vi "Test BB write read.vi"() -> ()   [LabVIEW 2021]
uses:
  typedef/Topic Full Names.ctl
  fc94ccf3-c4f9-4681-abcb-997b10467b18.vi
  1ecc9c55-0292-4034-a41c-db8078422293.vi
  9e8af28e-348a-4d52-b3a6-176f81345950.vi
  ff93d857-b347-4659-b587-d301aa5bbc46.vi
  d7d53fbf-e9ea-4da0-a5dc-3f6decd5c89f.vi
  386e704e-7c72-4735-ad53-a1b4597bfffc.vi
  aea694b6-2c48-4883-b1e6-448c91e8bea0.vi
  af7b2d98-0160-47b9-b2c8-6d5a41cd72f1.vi
  04c724ed-f4c4-49d6-b90b-59eac79b411c.vi
  10f2c807-d207-4ff9-b65f-d1b3e01e3914.vi
  96694315-c729-49e0-ae38-07976d2b01df.vi
  07ed32da-fde3-4ecc-a422-c66c6e158a99.vi
  5cbece44-eccb-42af-b590-0ccb7b3e0a3a.vi
  26da49ab-0f24-4915-9e5c-fae2186c0621.vi
  82d32cb3-3716-468c-9992-8dfaf92fc29f.vi
  0ce00b95-44ee-463c-baca-590a8846c1eb.vi
  5a159916-ffba-4323-afb6-8e2cf34b4672.vi
  0118180c-ae51-4c1e-a806-e67c93401480.vi
  9acccfa8-9bb2-4941-a38e-bb205dd59574.vi
  ab6a61a5-9c5f-449d-8423-f873c584b1ba.vi
  540d5d61-12e3-498b-9d40-879b6436794c.vi
  17e3f022-6cbe-4307-a055-1088f1a08aa5.vi
  b63f9921-ff80-4853-b2dc-f0cfe3ce2752.vi
  df38f484-dfd4-40f9-b9a1-491e45d6069d.vi
  dabef161-ca45-40be-b185-d2158fafdac9.vi
  599458bd-4083-4966-a6e9-0ee856bb8018.vi
  f13160dd-4d28-4d65-9fc8-a661e616088f.vi
  2429a5ee-c682-4303-b56b-a50622380fa0.vi
  c451a5a5-bbd7-4334-95d0-190131a98318.vi
  4afb852e-2286-42e1-bd7d-983000913123.vi
  c331ddf7-6c60-4b7b-82e2-165266058c85.vi
  989f7903-0cec-405a-8fc5-4e05a1e3b823.vi
  3f8d1f86-cf74-40ec-b4a0-b5d2f462e92c.vi
  c2603ed1-ff0f-47d7-9edf-26bf5f6ef7d4.vi
  9dc61f32-c8b2-401f-b4c2-5e38d3c4ff08.vi
  f2a7571f-032b-4f55-a724-f4471c08458c.vi
  dc893c51-4d2e-4bb4-b285-f4d4203b9537.vi
  91a0fbaa-2358-4159-8e72-b3850ae0b459.vi
  54bee8c1-0067-4be9-af3e-190d85fa807a.vi
  b4ab5d2e-a320-4709-8a65-b849ff6d5eac.vi
  c90ed56e-a4fb-44b1-b21c-7cee833b7fc2.vi
  8dfab18a-ac58-41df-a961-e3b183f267b1.vi
  6d6d06d4-fd38-4af0-8f86-16f866c4358f.vi
  70f752b6-94b3-46bc-87c5-c5551f755e49.vi
  87693e93-dc1b-4689-9420-073608a864a2.vi
  d23bcab6-9216-4072-ab24-334b80493afe.vi
  13594309-f9d5-44d8-84db-906724c8aeb8.vi
  5b121a18-a7f8-444b-bf3c-19de00dea731.vi
  b678fec2-0823-4dac-b98e-1ea96459124d.vi
  421e2864-b975-4d6e-8dba-970c1d659c6b.vi
  83d6945f-6206-48db-ba34-1315ddcf8622.vi
  334fafdd-3c45-415d-86a5-5c46786f1213.vi
  bdeeffe2-7481-4f0c-a63b-1c279b4d539b.vi
  daf0490c-48a1-49ff-a818-56076b47f53a.vi
  6d140309-082e-4568-9266-a5523fd3356c.vi
  cd00a663-0ed0-4c1c-bf6f-1e92360d99b7.vi
  0e6f1a11-abca-4238-a699-ce8b92277205.vi
  08820cd5-e149-4070-b260-5d58bdcecb90.vi
  8688fec4-49dd-4baa-ba4f-355704276364.vi
  62f858e5-9e8a-46a7-a3e9-f0995d3fb264.vi
  08794ecb-60ec-43ee-b589-61fe16b07a23.vi
  29a63749-4c43-41a6-a3ab-cfd97f2cae72.vi
  19342fc4-a6b3-4ce5-a15c-c0c74d8c0e55.vi
  0190af3f-4f2e-4064-95c6-6e90d87b853f.vi
  c9e0bfd6-1a21-40a0-b211-991072438108.vi
  849b2bb5-713d-46b1-af3e-8376bcd0ab32.vi
  SubVIs/Get Path.vi
  SubVIs/Convert Error.vi
  fc94ccf3-c4f9-4681-abcb-997b10467b18.vi/f164bb55-fadc-406a-97d8-e3295a396b46.vi
  SubVIs/Add Error.vi
  Refnum/BB from Refnum.vi
  Refnum/BB Writer to Refnum.vi
  <vilib>/CIF Foundation/CIF Utilities/File/File/File Not Found Error Update.vi
  1ecc9c55-0292-4034-a41c-db8078422293.vi/15451e88-64ef-462d-9cc0-58968935b893.vi
  Refnum/BB Reader to Refnum.vi
  Refnum/BB Writer from Refnum.vi
  Refnum/BB Reader from Refnum.vi
  386e704e-7c72-4735-ad53-a1b4597bfffc.vi/f164bb55-fadc-406a-97d8-e3295a396b46.vi
  aea694b6-2c48-4883-b1e6-448c91e8bea0.vi/15451e88-64ef-462d-9cc0-58968935b893.vi
  96694315-c729-49e0-ae38-07976d2b01df.vi/3bd89bd1-b605-4b55-aa60-227046f12b11.vi
  07ed32da-fde3-4ecc-a422-c66c6e158a99.vi/bd005753-9160-49ee-ba23-7aa8055d86ff.vi
  0ce00b95-44ee-463c-baca-590a8846c1eb.vi/3bd89bd1-b605-4b55-aa60-227046f12b11.vi
  5a159916-ffba-4323-afb6-8e2cf34b4672.vi/bd005753-9160-49ee-ba23-7aa8055d86ff.vi
  540d5d61-12e3-498b-9d40-879b6436794c.vi/f164bb55-fadc-406a-97d8-e3295a396b46.vi
  17e3f022-6cbe-4307-a055-1088f1a08aa5.vi/15451e88-64ef-462d-9cc0-58968935b893.vi
  f13160dd-4d28-4d65-9fc8-a661e616088f.vi/f164bb55-fadc-406a-97d8-e3295a396b46.vi
  2429a5ee-c682-4303-b56b-a50622380fa0.vi/15451e88-64ef-462d-9cc0-58968935b893.vi
  3f8d1f86-cf74-40ec-b4a0-b5d2f462e92c.vi/f164bb55-fadc-406a-97d8-e3295a396b46.vi
  c2603ed1-ff0f-47d7-9edf-26bf5f6ef7d4.vi/15451e88-64ef-462d-9cc0-58968935b893.vi
  dc893c51-4d2e-4bb4-b285-f4d4203b9537.vi/f164bb55-fadc-406a-97d8-e3295a396b46.vi
  91a0fbaa-2358-4159-8e72-b3850ae0b459.vi/15451e88-64ef-462d-9cc0-58968935b893.vi
  c90ed56e-a4fb-44b1-b21c-7cee833b7fc2.vi/f164bb55-fadc-406a-97d8-e3295a396b46.vi
  8dfab18a-ac58-41df-a961-e3b183f267b1.vi/15451e88-64ef-462d-9cc0-58968935b893.vi
  87693e93-dc1b-4689-9420-073608a864a2.vi/3bd89bd1-b605-4b55-aa60-227046f12b11.vi
  Refnum/BB Raw Reader to Refnum.vi
  Refnum/BB Raw Reader from Refnum.vi
  13594309-f9d5-44d8-84db-906724c8aeb8.vi/c28b0ead-42ad-4072-80a2-aca7f2bd7ce3.vi
  13594309-f9d5-44d8-84db-906724c8aeb8.vi/48104490-ec73-4168-8754-ff252ec03617.vi
  <vilib>/CIF Foundation/CIF Utilities/DataTypes/SubVIs/DataTypes Error.vi
  13594309-f9d5-44d8-84db-906724c8aeb8.vi/543c0f61-77eb-4f29-b175-1688c1700ba4.vi
  b678fec2-0823-4dac-b98e-1ea96459124d.vi/f164bb55-fadc-406a-97d8-e3295a396b46.vi
  421e2864-b975-4d6e-8dba-970c1d659c6b.vi/15451e88-64ef-462d-9cc0-58968935b893.vi
  daf0490c-48a1-49ff-a818-56076b47f53a.vi/f164bb55-fadc-406a-97d8-e3295a396b46.vi
  6d140309-082e-4568-9266-a5523fd3356c.vi/15451e88-64ef-462d-9cc0-58968935b893.vi
  8688fec4-49dd-4baa-ba4f-355704276364.vi/f164bb55-fadc-406a-97d8-e3295a396b46.vi
  62f858e5-9e8a-46a7-a3e9-f0995d3fb264.vi/3bd89bd1-b605-4b55-aa60-227046f12b11.vi
  08794ecb-60ec-43ee-b589-61fe16b07a23.vi/bd005753-9160-49ee-ba23-7aa8055d86ff.vi
  Refnum/BB Raw Writer to Refnum.vi
  Refnum/BB Raw Writer from Refnum.vi
  <vilib>/Utility/error.llb/Trim Whitespace.vi
  SubVIs/Add Error Core.vi
  <vilib>/CIF Foundation/CIF Utilities/DataTypes/Utilities/Get Element Info of Variant.vi
  SubVIs/Get Type String.vi
  <vilib>/CIF Foundation/CIF Utilities/DataTypes/Utilities/Get JSON Descriptor of Variant.vi
  SubVIs/Convert Error Core.vi
  <vilib>/CIF Foundation/CIF Utilities/File/SubVIs/File Not Found Error Core.vi
  <vilib>/CIF Foundation/CIF Utilities/DataTypes/SubVIs/DataTypes Error Core.vi
  Iceoryx.lvlib
panel:
  out "status":string
  out "pass":bool
  out "error out":errorcluster
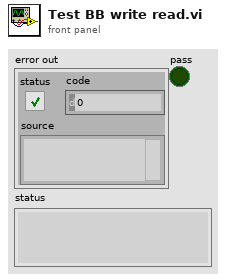
[diagram p1: front panel]
types:
  T1 = typedef "Iceoryx.lvlib/Topic Full Names.ctl" = cluster{"BlackBoard":string, "Topic":string, "Type Override":string}
  T2 = cluster{"U16":u16, "test_I32":i32, bool, "embedded":cluster{dbl, "bool":bool}}
  T3 = typedef "Iceoryx.lvlib/BB Refnum.ctl" = cluster{"refnum":u64, "BB":enum8{"bb"}}
  T4 = typedef "Iceoryx.lvlib/BB Writer Refnum.ctl" = cluster{"refnum":u64, "BB Writer":enum8{"bb_writer"}}
  T5 = typedef "Iceoryx.lvlib/BB Reader Refnum.ctl" = cluster{"refnum":u64, "BB Reader":enum8{"bb_reader"}}
  T6 = cluster{"U16":u16, "I32":i32, bool, "embedded":cluster{dbl, "bool":bool}}
  T7 = typedef "Iceoryx.lvlib/BB Raw Reader Refnum.ctl" = cluster{"refnum":u64, "BB Raw Reader":enum8{"bb_raw_reader"}}
  T8 = typedef "Iceoryx.lvlib/BB Raw Writer Refnum.ctl" = cluster{"refnum":u64, "BB Raw Writer":enum8{"bb_raw_writer"}}
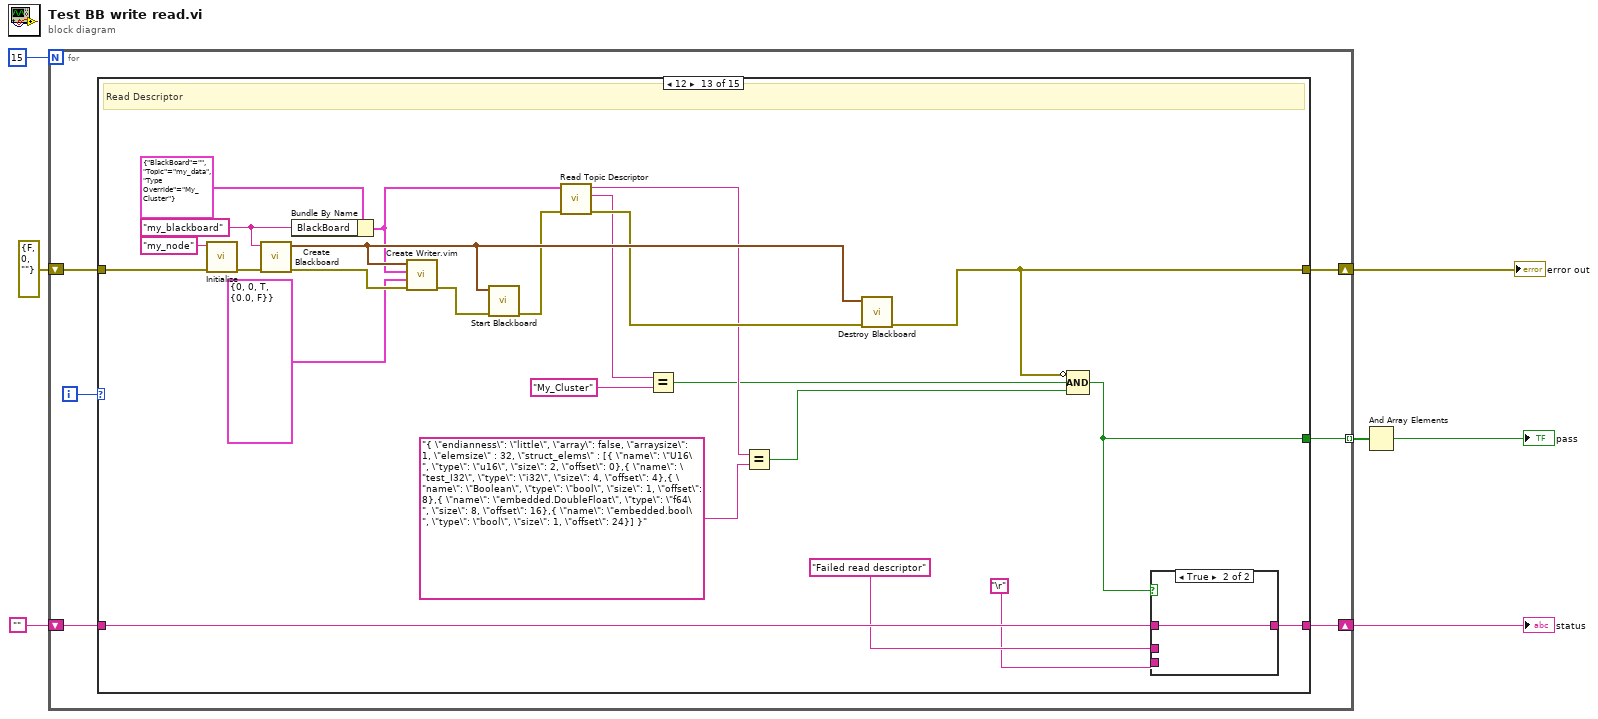
[diagram p0: block diagram]
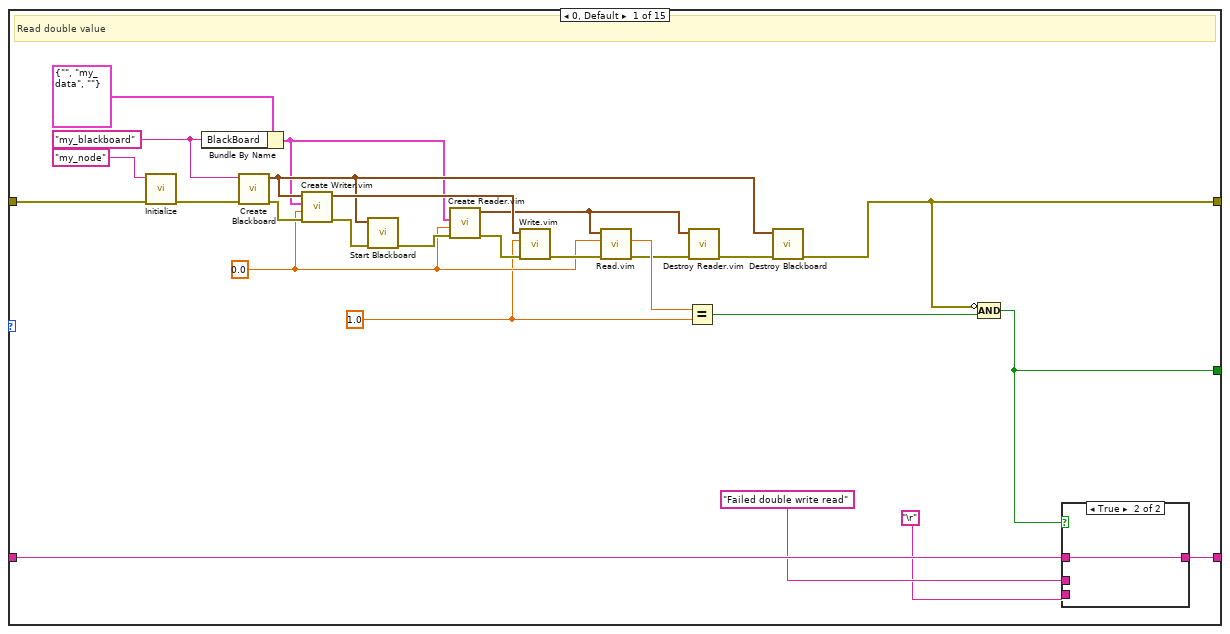
[diagram p2: hidden frame]
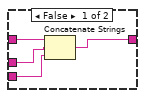
[diagram p3: hidden frame]
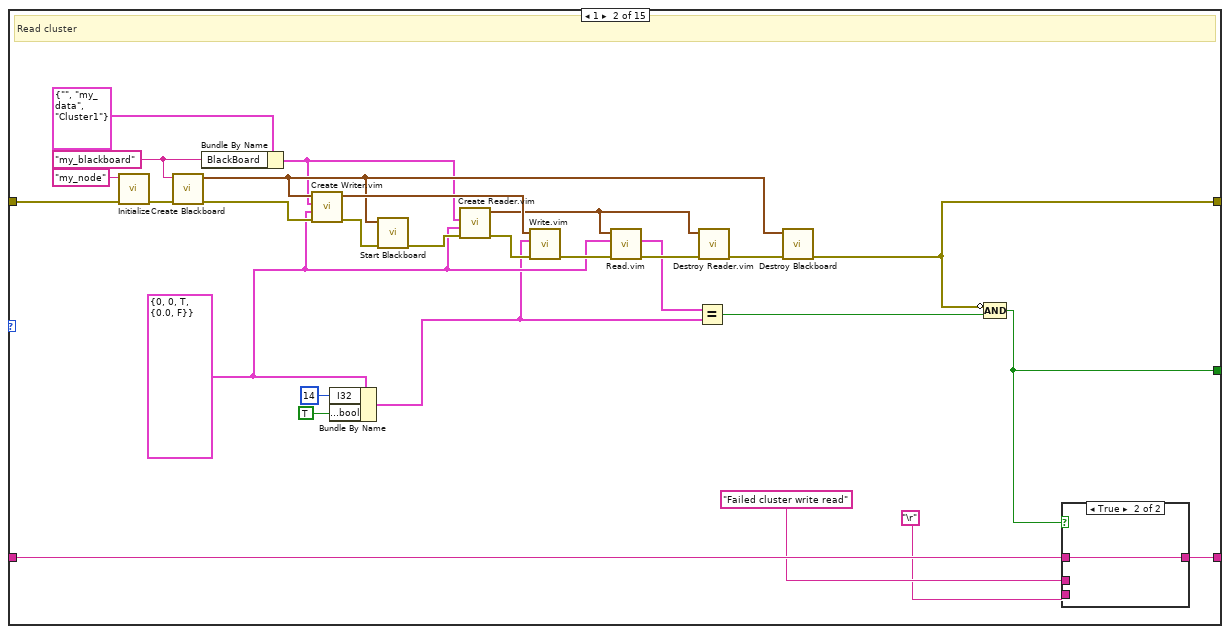
[diagram p4: hidden frame]
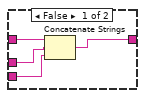
[diagram p5: hidden frame]
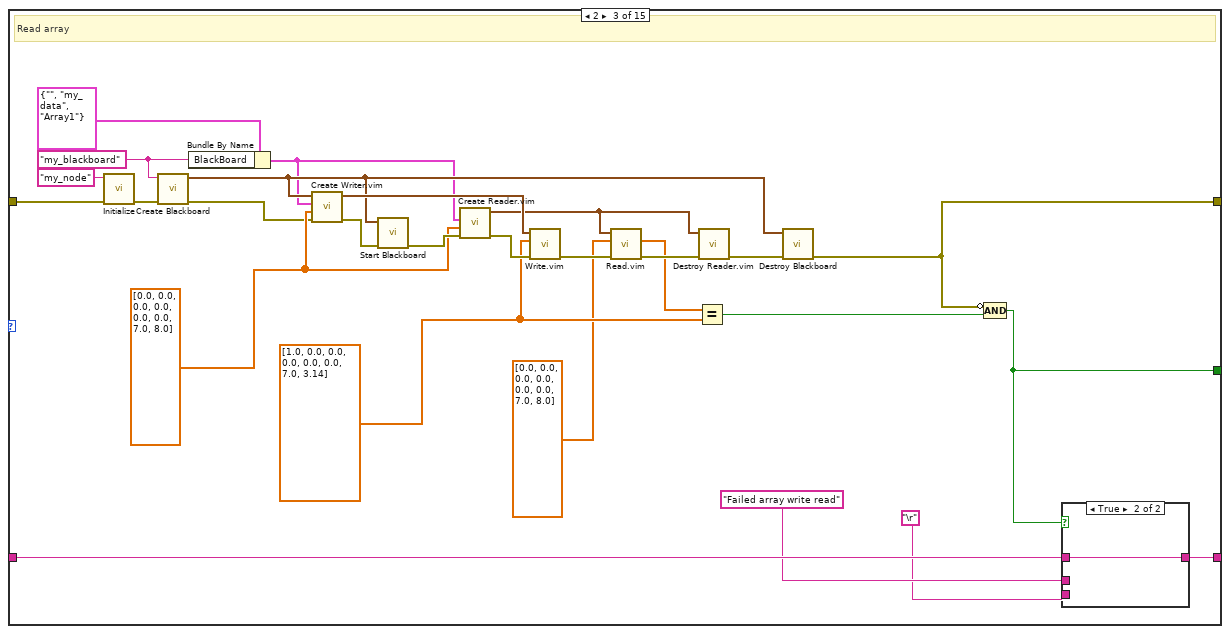
[diagram p6: hidden frame]
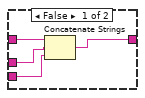
[diagram p7: hidden frame]
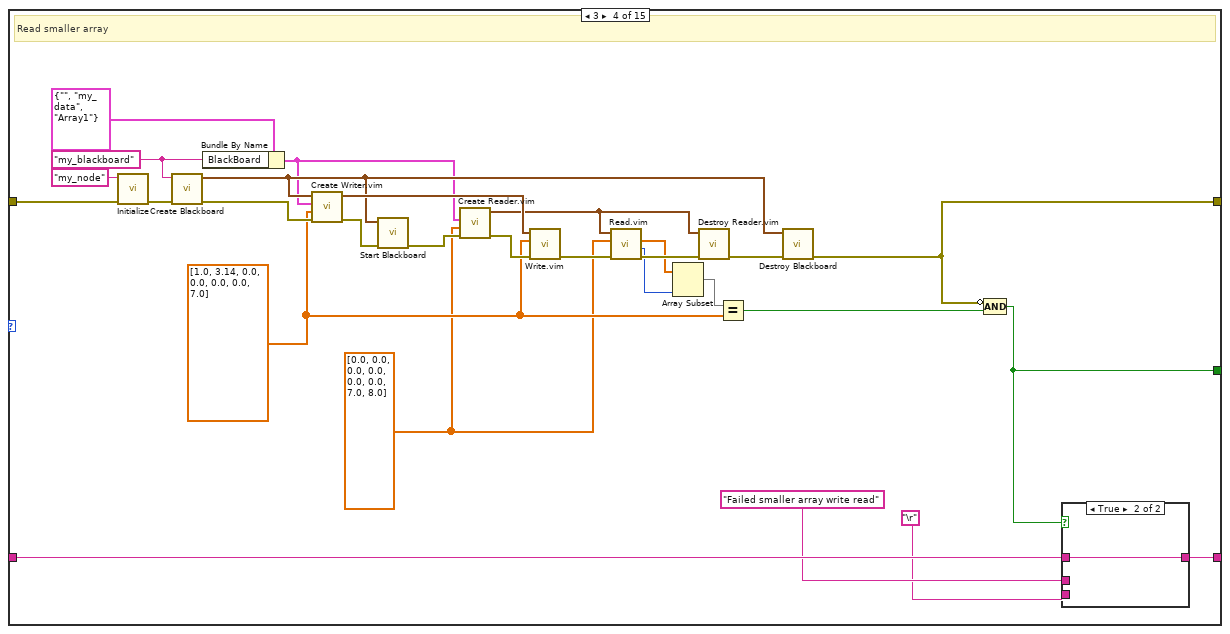
[diagram p8: hidden frame]
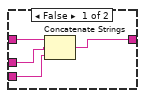
[diagram p9: hidden frame]
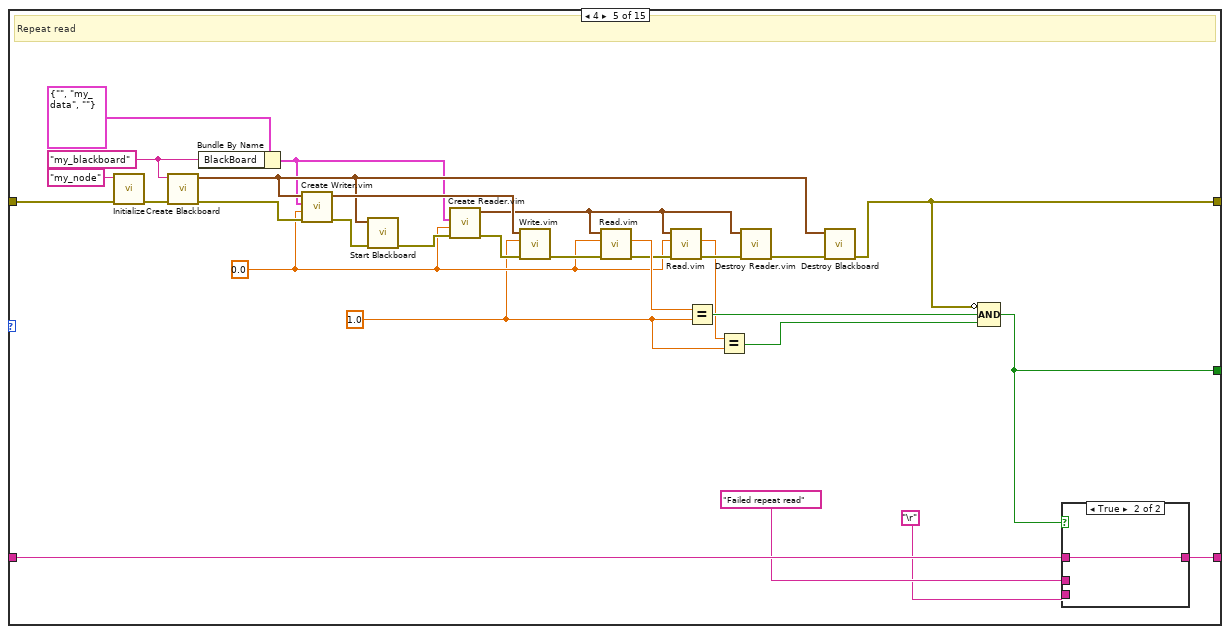
[diagram p10: hidden frame]
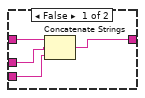
[diagram p11: hidden frame]
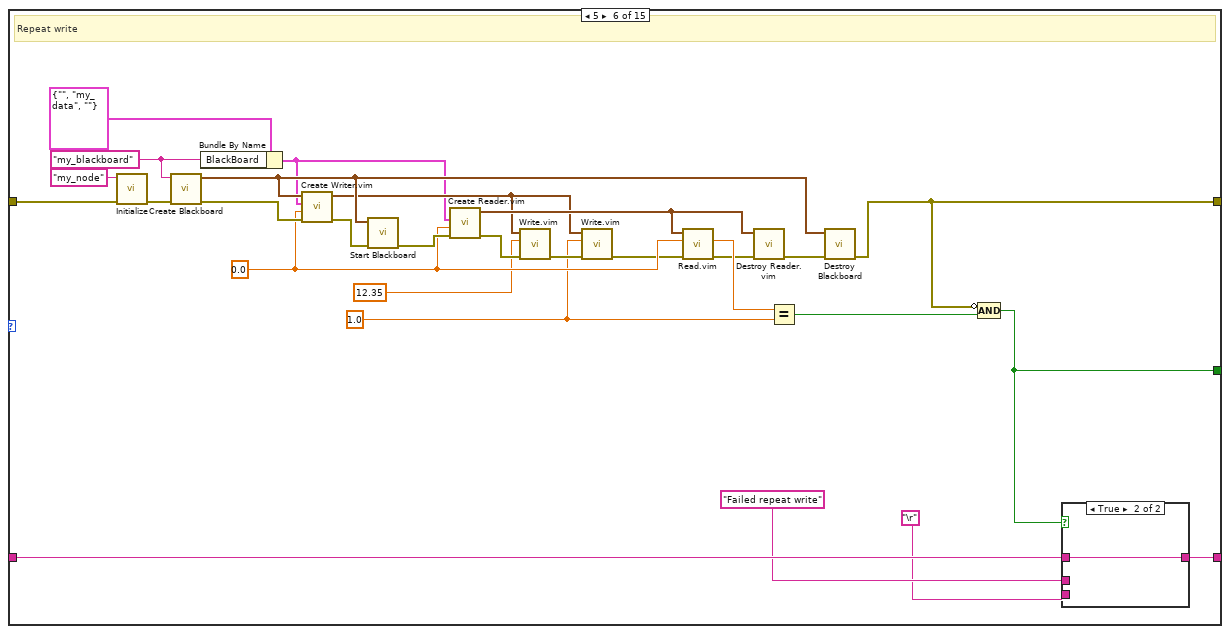
[diagram p12: hidden frame]
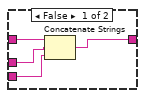
[diagram p13: hidden frame]
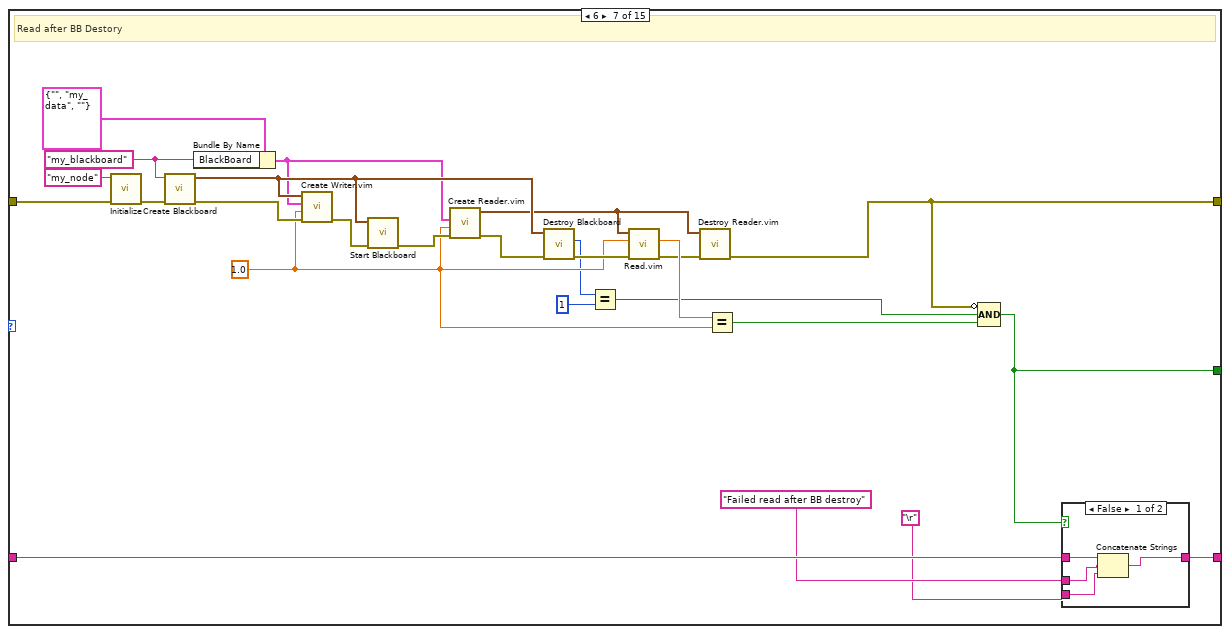
[diagram p14: hidden frame]
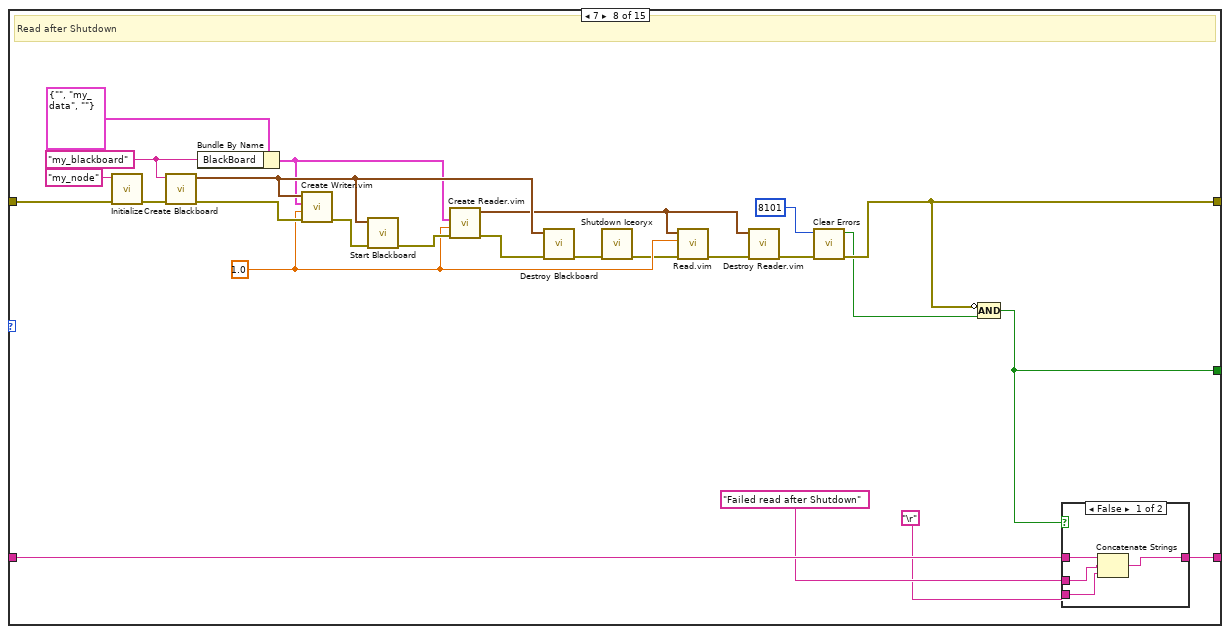
[diagram p16: hidden frame]
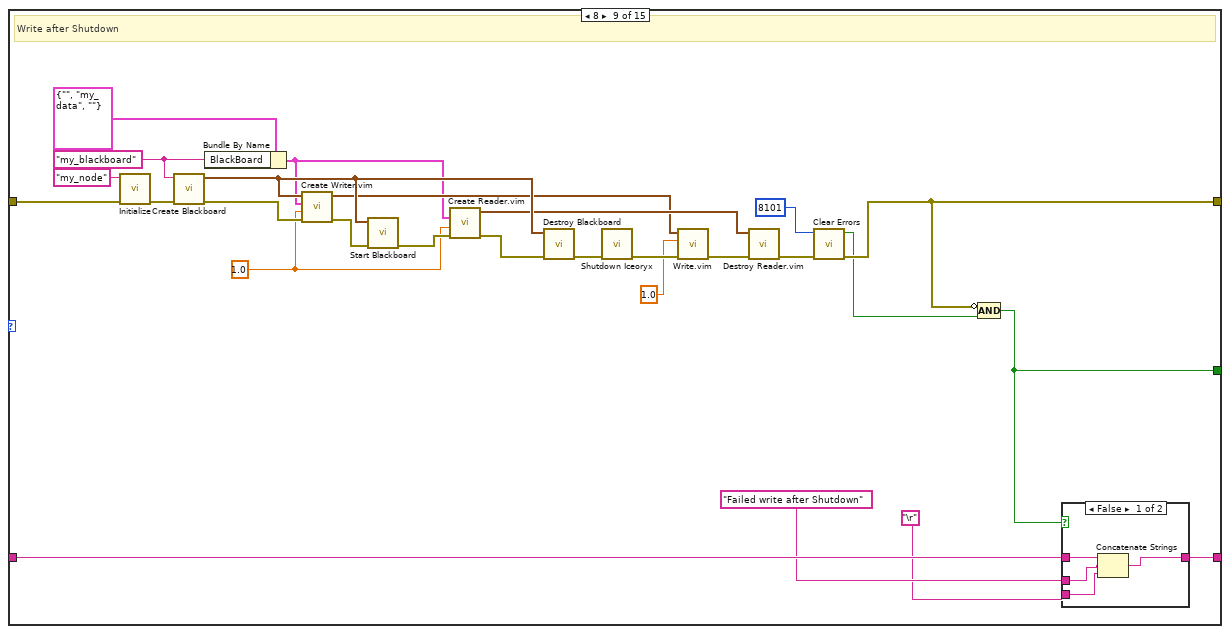
[diagram p18: hidden frame]
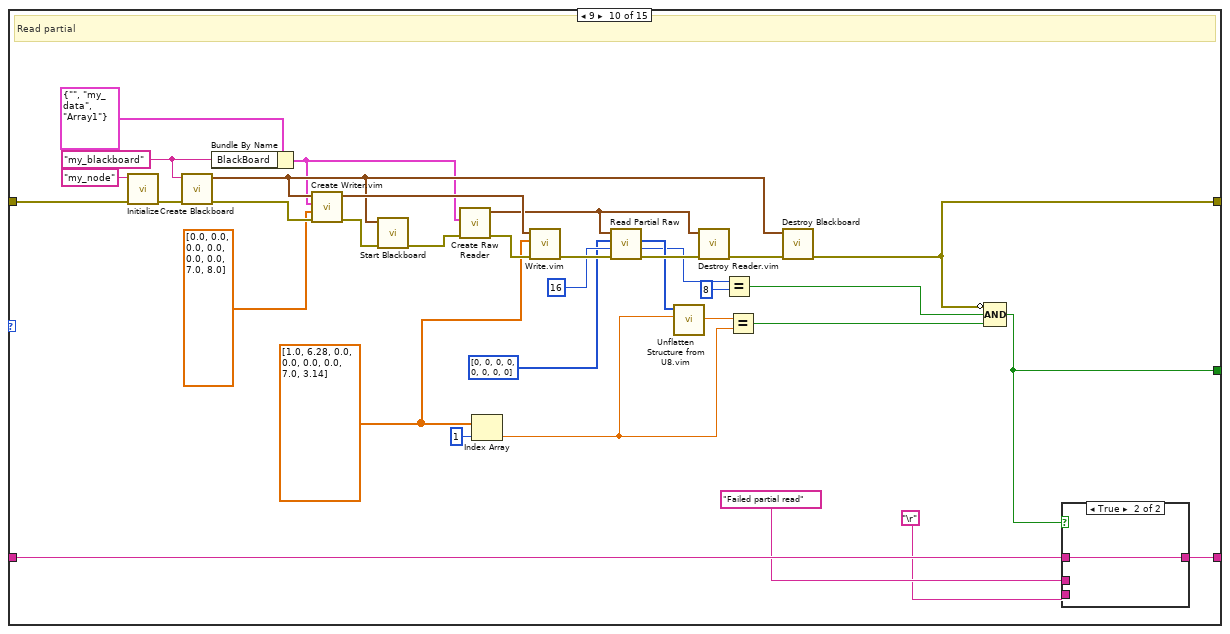
[diagram p20: hidden frame]
diagram:
  n1 = for {
    N: 15 -> [_]
    tunnel: [w13] -> w7 mode=indexing
    shift-right: [w11] -> w3
    shift-left: "" -> [w12]
    shift-right: [w10] -> w1
    shift-left: errorcluster {"status"=FALSE, "code"=0, "source"=""} ("error out") -> [w9]
    i -> [w8]
    n2 = case shown="12" w8 {
      tunnel: [w35 w48 w86 w118 w167 w200 w231 w261 w293 w318 w366 w403 w432 w458 w485] -> w13
      tunnel: w12 -> [w39 w72 w104 w137 w171 w204 w235 w265 w297 w336 w370 w407 w436 w471 w503]
      tunnel: [w38 w71 w103 w136 w170 w203 w234 w264 w296 w335 w369 w406 w435 w470 w502] -> w11
      tunnel: [w19 w53 w87 w119 w153 w188 w219 w246 w278 w319 w350 w389 w425 w459 w486] -> w10
      tunnel: w9 -> [w32 w54 w88 w120 w164 w197 w229 w259 w291 w320 w363 w400 w430 w460 w487]
      frame 0, Default {
        w21 = 0.0
        w14 = 1.0
        w16 = "my_blackboard" ("Blackboard name")
        # "Read double value"
        n3 = call "Initialize.vi"("error in (no error)"=w32, "Node name"="my_node") -> ("error out"=w33:errorcluster)  [unwired: 9 in]
        n4 = Bundle By Name(cluster=T1 {"BlackBoard"="", "Topic"="my_data", "Type Override"=""} ("Topic Full Names"), "BlackBoard"=w16) -> (w15:T1)
        n5 = call "Create Blackboard.vi"("error in (no error)"=w33, "Blackboard name"=w16) -> ("error out"=w30:errorcluster, "Blackboard Reference"=w22:T3)  [unwired: 8 in]
        n6 = call "Create Writer.vim"("error in (no error)"=w30, "Data"=w21, "Topic Name"=w15, "BlackBoard Reference"=w22) -> ("error out"=w31:errorcluster, "Writer Reference"=w24:T4)  [unwired: 5 in, 1 out]
        n7 = call "Start Blackboard.vi"("error in (no error)"=w31, "Blackboard Reference"=w22) -> ("error out"=w29:errorcluster)  [unwired: 9 in]
        n8 = call "Create Reader.vim"("error in (no error)"=w29, "Data Type"=w21, "Topic Name"=w15) -> ("error out"=w28:errorcluster, "Reader Reference"=w23:T5)  [unwired: 6 in, 1 out]
        n9 = call "Write.vim"("error in (no error)"=w28, "Data In"=w14, "Writer Reference"=w24) -> ("error out"=w27:errorcluster)  [unwired: 7 in, 1 out]
        n10 = call "Read.vim"("error in (no error)"=w27, "Data In"=w21, "Reader Reference"=w23) -> ("error out"=w17:errorcluster, "Data Out"=w20:dbl)  [unwired: 6 in, 1 out]
        n11 = Equal?(x=w20, y=w14) -> (x = y?=w34:bool)
        n12 = call "Destroy Reader.vim"("error in (no error)"=w17, "Reader Reference"=w23) -> ("error out"=w26:errorcluster)  [unwired: 9 in]
        n13 = call "Destroy Blackboard.vi"("error in (no error)"=w26, "Blackboard Reference"=w22) -> ("error out"=w19:errorcluster)  [unwired: 8 in, 1 out]
        n14 = Compound Arithmetic op=AND(invert w19, w34) -> (w35:bool)
        n15 = case shown="True" w35 {
          tunnel: w39 -> [w43 w44]
          tunnel: [w40 w44] -> w38
          tunnel: "Failed double write read" -> [w42 _]
          tunnel: "\r" -> [w41 _]
          frame False {
            n16 = Concatenate Strings(w43, w42, w41) -> (w40:string)
          }
          frame True {
          }
        }
      }
      frame 1 {
        w50 = T6 {"U16"=0, "I32"=0, TRUE, "embedded"={0.0, "bool"=FALSE}}
        w47 = "my_blackboard" ("Blackboard name")
        # "Read cluster"
        n17 = call "Initialize.vi"("error in (no error)"=w54, "Node name"="my_node") -> ("error out"=w67:errorcluster)  [unwired: 9 in]
        n18 = call "Create Blackboard.vi"("error in (no error)"=w67, "Blackboard name"=w47) -> ("error out"=w65:errorcluster, "Blackboard Reference"=w56:T3)  [unwired: 8 in]
        n19 = Bundle By Name(cluster=T1 {"BlackBoard"="", "Topic"="my_data", "Type Override"="Cluster1"} ("Topic Full Names"), "BlackBoard"=w47) -> (w45:T1)
        n20 = call "Create Writer.vim"("error in (no error)"=w65, "Data"=w50, "Topic Name"=w45, "BlackBoard Reference"=w56) -> ("error out"=w66:errorcluster, "Writer Reference"=w58:T4)  [unwired: 5 in, 1 out]
        n21 = Bundle By Name(cluster=w50, "I32"=14, "embedded.bool"=TRUE) -> (w49:T6)
        n22 = call "Start Blackboard.vi"("error in (no error)"=w66, "Blackboard Reference"=w56) -> ("error out"=w64:errorcluster)  [unwired: 9 in]
        n23 = call "Create Reader.vim"("error in (no error)"=w64, "Data Type"=w50, "Topic Name"=w45) -> ("error out"=w63:errorcluster, "Reader Reference"=w57:T5)  [unwired: 6 in, 1 out]
        n24 = call "Write.vim"("error in (no error)"=w63, "Data In"=w49, "Writer Reference"=w58) -> ("error out"=w62:errorcluster)  [unwired: 7 in, 1 out]
        n25 = call "Read.vim"("error in (no error)"=w62, "Data In"=w50, "Reader Reference"=w57) -> ("error out"=w61:errorcluster, "Data Out"=w55:T6)  [unwired: 6 in, 1 out]
        n26 = Equal?(x=w55, y=w49) -> (x = y?=w68:bool)
        n27 = call "Destroy Reader.vim"("error in (no error)"=w61, "Reader Reference"=w57) -> ("error out"=w60:errorcluster)  [unwired: 9 in]
        n28 = call "Destroy Blackboard.vi"("error in (no error)"=w60, "Blackboard Reference"=w56) -> ("error out"=w53:errorcluster)  [unwired: 8 in, 1 out]
        n29 = Compound Arithmetic op=AND(invert w53, w68) -> (w48:bool)
        n30 = case shown="True" w48 {
          tunnel: w72 -> [w76 w77]
          tunnel: [w73 w77] -> w71
          tunnel: "Failed cluster write read" -> [w75 _]
          tunnel: "\r" -> [w74 _]
          frame False {
            n31 = Concatenate Strings(w76, w75, w74) -> (w73:string)
          }
          frame True {
          }
        }
      }
      frame 2 {
        w84 = dbl[] [1.0, 0.0, 0.0, 0.0, 0.0, 0.0, 7.0, 3.14]
        w85 = dbl[] [0.0, 0.0, 0.0, 0.0, 0.0, 0.0, 7.0, 8.0]
        w80 = "my_blackboard" ("Blackboard name")
        # "Read array"
        n32 = call "Initialize.vi"("error in (no error)"=w88, "Node name"="my_node") -> ("error out"=w99:errorcluster)  [unwired: 9 in]
        n33 = call "Create Blackboard.vi"("error in (no error)"=w99, "Blackboard name"=w80) -> ("error out"=w79:errorcluster, "Blackboard Reference"=w89:T3)  [unwired: 8 in]
        n34 = Bundle By Name(cluster=T1 {"BlackBoard"="", "Topic"="my_data", "Type Override"="Array1"} ("Topic Full Names"), "BlackBoard"=w80) -> (w78:T1)
        n35 = call "Create Writer.vim"("error in (no error)"=w79, "Data"=w85, "Topic Name"=w78, "BlackBoard Reference"=w89) -> ("error out"=w98:errorcluster, "Writer Reference"=w91:T4)  [unwired: 5 in, 1 out]
        n36 = call "Start Blackboard.vi"("error in (no error)"=w98, "Blackboard Reference"=w89) -> ("error out"=w97:errorcluster)  [unwired: 9 in]
        n37 = call "Create Reader.vim"("error in (no error)"=w97, "Data Type"=w85, "Topic Name"=w78) -> ("error out"=w96:errorcluster, "Reader Reference"=w90:T5)  [unwired: 6 in, 1 out]
        n38 = call "Write.vim"("error in (no error)"=w96, "Data In"=w84, "Writer Reference"=w91) -> ("error out"=w95:errorcluster)  [unwired: 7 in, 1 out]
        n39 = call "Read.vim"("error in (no error)"=w95, "Data In"=dbl[] [0.0, 0.0, 0.0, 0.0, 0.0, 0.0, 7.0, 8.0], "Reader Reference"=w90) -> ("error out"=w94:errorcluster, "Data Out"=w83:dbl[])  [unwired: 6 in, 1 out]
        n40 = Equal?(x=w83, y=w84) -> (x = y?=w100:bool)
        n41 = call "Destroy Reader.vim"("error in (no error)"=w94, "Reader Reference"=w90) -> ("error out"=w93:errorcluster)  [unwired: 9 in]
        n42 = call "Destroy Blackboard.vi"("error in (no error)"=w93, "Blackboard Reference"=w89) -> ("error out"=w87:errorcluster)  [unwired: 8 in, 1 out]
        n43 = Compound Arithmetic op=AND(invert w87, w100) -> (w86:bool)
        n44 = case shown="True" w86 {
          tunnel: w104 -> [w108 w109]
          tunnel: [w105 w109] -> w103
          tunnel: "Failed array write read" -> [w107 _]
          tunnel: "\r" -> [w106 _]
          frame False {
            n45 = Concatenate Strings(w108, w107, w106) -> (w105:string)
          }
          frame True {
          }
        }
      }
      frame 3 {
        w116 = dbl[] [0.0, 0.0, 0.0, 0.0, 0.0, 0.0, 7.0, 8.0]
        w117 = dbl[] [1.0, 3.14, 0.0, 0.0, 0.0, 0.0, 7.0]
        w111 = "my_blackboard" ("Blackboard name")
        # "Read smaller array"
        n46 = call "Initialize.vi"("error in (no error)"=w120, "Node name"="my_node") -> ("error out"=w132:errorcluster)  [unwired: 9 in]
        n47 = call "Create Blackboard.vi"("error in (no error)"=w132, "Blackboard name"=w111) -> ("error out"=w130:errorcluster, "Blackboard Reference"=w121:T3)  [unwired: 8 in]
        n48 = Bundle By Name(cluster=T1 {"BlackBoard"="", "Topic"="my_data", "Type Override"="Array1"} ("Topic Full Names"), "BlackBoard"=w111) -> (w110:T1)
        n49 = call "Create Writer.vim"("error in (no error)"=w130, "Data"=w117, "Topic Name"=w110, "BlackBoard Reference"=w121) -> ("error out"=w131:errorcluster, "Writer Reference"=w123:T4)  [unwired: 5 in, 1 out]
        n50 = call "Start Blackboard.vi"("error in (no error)"=w131, "Blackboard Reference"=w121) -> ("error out"=w129:errorcluster)  [unwired: 9 in]
        n51 = call "Create Reader.vim"("error in (no error)"=w129, "Data Type"=w116, "Topic Name"=w110) -> ("error out"=w128:errorcluster, "Reader Reference"=w122:T5)  [unwired: 6 in, 1 out]
        n52 = call "Write.vim"("error in (no error)"=w128, "Data In"=w117, "Writer Reference"=w123) -> ("error out"=w127:errorcluster)  [unwired: 7 in, 1 out]
        n53 = call "Read.vim"("error in (no error)"=w127, "Data In"=w116, "Reader Reference"=w122) -> ("error out"=w126:errorcluster, "Array Length"=w114:u32, "Data Out"=w115:dbl[])  [unwired: 6 in]
        n54 = Array Subset(array=w115, length=w114) -> (w113:dbl[])  [unwired: 1 in]
        n55 = call "Destroy Reader.vim"("error in (no error)"=w126, "Reader Reference"=w122) -> ("error out"=w125:errorcluster)  [unwired: 9 in]
        n56 = Equal?(x=w113, y=w117) -> (x = y?=w133:bool)
        n57 = call "Destroy Blackboard.vi"("error in (no error)"=w125, "Blackboard Reference"=w121) -> ("error out"=w119:errorcluster)  [unwired: 8 in, 1 out]
        n58 = Compound Arithmetic op=AND(invert w119, w133) -> (w118:bool)
        n59 = case shown="True" w118 {
          tunnel: w137 -> [w141 w142]
          tunnel: [w138 w142] -> w136
          tunnel: "Failed smaller array write read" -> [w140 _]
          tunnel: "\r" -> [w139 _]
          frame False {
            n60 = Concatenate Strings(w141, w140, w139) -> (w138:string)
          }
          frame True {
          }
        }
      }
      frame 4 {
        w149 = 0.0
        w143 = 1.0
        w146 = "my_blackboard" ("Blackboard name")
        # "Repeat read"
        n61 = call "Initialize.vi"("error in (no error)"=w164, "Node name"="my_node") -> ("error out"=w165:errorcluster)  [unwired: 9 in]
        n62 = call "Create Blackboard.vi"("error in (no error)"=w165, "Blackboard name"=w146) -> ("error out"=w162:errorcluster, "Blackboard Reference"=w155:T3)  [unwired: 8 in]
        n63 = Bundle By Name(cluster=T1 {"BlackBoard"="", "Topic"="my_data", "Type Override"=""} ("Topic Full Names"), "BlackBoard"=w146) -> (w145:T1)
        n64 = call "Create Writer.vim"("error in (no error)"=w162, "Data"=w149, "Topic Name"=w145, "BlackBoard Reference"=w155) -> ("error out"=w163:errorcluster, "Writer Reference"=w156:T4)  [unwired: 5 in, 1 out]
        n65 = call "Start Blackboard.vi"("error in (no error)"=w163, "Blackboard Reference"=w155) -> ("error out"=w161:errorcluster)  [unwired: 9 in]
        n66 = call "Create Reader.vim"("error in (no error)"=w161, "Data Type"=w149, "Topic Name"=w145) -> ("error out"=w160:errorcluster, "Reader Reference"=w150:T5)  [unwired: 6 in, 1 out]
        n67 = call "Write.vim"("error in (no error)"=w160, "Data In"=w143, "Writer Reference"=w156) -> ("error out"=w159:errorcluster)  [unwired: 7 in, 1 out]
        n68 = call "Read.vim"("error in (no error)"=w159, "Data In"=w149, "Reader Reference"=w150) -> ("error out"=w152:errorcluster, "Data Out"=w154:dbl)  [unwired: 6 in, 1 out]
        n69 = call "Read.vim"("error in (no error)"=w152, "Data In"=w149, "Reader Reference"=w150) -> ("error out"=w151:errorcluster, "Data Out"=w148:dbl)  [unwired: 6 in, 1 out]
        n70 = Equal?(x=w154, y=w143) -> (x = y?=w166:bool)
        n71 = Equal?(x=w148, y=w143) -> (x = y?=w147:bool)
        n72 = call "Destroy Reader.vim"("error in (no error)"=w151, "Reader Reference"=w150) -> ("error out"=w158:errorcluster)  [unwired: 9 in]
        n73 = call "Destroy Blackboard.vi"("error in (no error)"=w158, "Blackboard Reference"=w155) -> ("error out"=w153:errorcluster)  [unwired: 8 in, 1 out]
        n74 = Compound Arithmetic op=AND(invert w153, w166, w147) -> (w167:bool)
        n75 = case shown="True" w167 {
          tunnel: w171 -> [w175 w176]
          tunnel: [w172 w176] -> w170
          tunnel: "Failed repeat read" -> [w174 _]
          tunnel: "\r" -> [w173 _]
          frame False {
            n76 = Concatenate Strings(w175, w174, w173) -> (w172:string)
          }
          frame True {
          }
        }
      }
      frame 5 {
        w186 = 0.0
        w177 = 1.0
        w179 = "my_blackboard" ("Blackboard name")
        # "Repeat write"
        n77 = call "Initialize.vi"("error in (no error)"=w197, "Node name"="my_node") -> ("error out"=w198:errorcluster)  [unwired: 9 in]
        n78 = call "Create Blackboard.vi"("error in (no error)"=w198, "Blackboard name"=w179) -> ("error out"=w195:errorcluster, "Blackboard Reference"=w190:T3)  [unwired: 8 in]
        n79 = Bundle By Name(cluster=T1 {"BlackBoard"="", "Topic"="my_data", "Type Override"=""} ("Topic Full Names"), "BlackBoard"=w179) -> (w178:T1)
        n80 = call "Create Writer.vim"("error in (no error)"=w195, "Data"=w186, "Topic Name"=w178, "BlackBoard Reference"=w190) -> ("error out"=w196:errorcluster, "Writer Reference"=w181:T4)  [unwired: 5 in, 1 out]
        n81 = call "Start Blackboard.vi"("error in (no error)"=w196, "Blackboard Reference"=w190) -> ("error out"=w194:errorcluster)  [unwired: 9 in]
        n82 = call "Create Reader.vim"("error in (no error)"=w194, "Data Type"=w186, "Topic Name"=w178) -> ("error out"=w193:errorcluster, "Reader Reference"=w187:T5)  [unwired: 6 in, 1 out]
        n83 = call "Write.vim"("error in (no error)"=w193, "Data In"=12.35, "Writer Reference"=w181) -> ("error out"=w184:errorcluster)  [unwired: 7 in, 1 out]
        n84 = call "Write.vim"("error in (no error)"=w184, "Data In"=w177, "Writer Reference"=w181) -> ("error out"=w183:errorcluster)  [unwired: 7 in, 1 out]
        n85 = call "Read.vim"("error in (no error)"=w183, "Data In"=w186, "Reader Reference"=w187) -> ("error out"=w185:errorcluster, "Data Out"=w189:dbl)  [unwired: 6 in, 1 out]
        n86 = call "Destroy Reader.vim"("error in (no error)"=w185, "Reader Reference"=w187) -> ("error out"=w192:errorcluster)  [unwired: 9 in]
        n87 = Equal?(x=w189, y=w177) -> (x = y?=w199:bool)
        n88 = call "Destroy Blackboard.vi"("error in (no error)"=w192, "Blackboard Reference"=w190) -> ("error out"=w188:errorcluster)  [unwired: 8 in, 1 out]
        n89 = Compound Arithmetic op=AND(invert w188, w199) -> (w200:bool)
        n90 = case shown="True" w200 {
          tunnel: w204 -> [w208 w209]
          tunnel: [w205 w209] -> w203
          tunnel: "Failed repeat write" -> [w207 _]
          tunnel: "\r" -> [w206 _]
          frame False {
            n91 = Concatenate Strings(w208, w207, w206) -> (w205:string)
          }
          frame True {
          }
        }
      }
      frame 6 {
        w217 = 1.0
        w211 = "my_blackboard" ("Blackboard name")
        # "Read after BB Destory"
        n92 = call "Initialize.vi"("error in (no error)"=w229, "Node name"="my_node") -> ("error out"=w230:errorcluster)  [unwired: 9 in]
        n93 = call "Create Blackboard.vi"("error in (no error)"=w230, "Blackboard name"=w211) -> ("error out"=w227:errorcluster, "Blackboard Reference"=w224:T3)  [unwired: 8 in]
        n94 = Bundle By Name(cluster=T1 {"BlackBoard"="", "Topic"="my_data", "Type Override"=""} ("Topic Full Names"), "BlackBoard"=w211) -> (w210:T1)
        n95 = call "Create Writer.vim"("error in (no error)"=w227, "Data"=w217, "Topic Name"=w210, "BlackBoard Reference"=w224) -> ("error out"=w228:errorcluster)  [unwired: 5 in, 2 out]
        n96 = call "Start Blackboard.vi"("error in (no error)"=w228, "Blackboard Reference"=w224) -> ("error out"=w226:errorcluster)  [unwired: 9 in]
        n97 = call "Create Reader.vim"("error in (no error)"=w226, "Data Type"=w217, "Topic Name"=w210) -> ("error out"=w220:errorcluster, "Reader Reference"=w222:T5)  [unwired: 6 in, 1 out]
        n98 = call "Destroy Blackboard.vi"("error in (no error)"=w220, "Blackboard Reference"=w224) -> ("error out"=w218:errorcluster, "readers_remaining"=w215:i32)  [unwired: 8 in]
        n99 = Equal?(x=w215, y=1) -> (x = y?=w213:bool)
        n100 = call "Read.vim"("error in (no error)"=w218, "Data In"=w217, "Reader Reference"=w222) -> ("error out"=w221:errorcluster, "Data Out"=w223:dbl)  [unwired: 6 in, 1 out]
        n101 = call "Destroy Reader.vim"("error in (no error)"=w221, "Reader Reference"=w222) -> ("error out"=w219:errorcluster)  [unwired: 9 in]
        n102 = Equal?(x=w223, y=w217) -> (x = y?=w216:bool)
        n103 = Compound Arithmetic op=AND(invert w219, w213, w216) -> (w231:bool)
        n104 = case shown="False" w231 {
          tunnel: w235 -> [w239 w240]
          tunnel: [w236 w240] -> w234
          tunnel: "Failed read after BB destroy" -> [w238 _]
          tunnel: "\r" -> [w237 _]
          frame False {
            n105 = Concatenate Strings(w239, w238, w237) -> (w236:string)
          }
          frame True {
          }
        }
      }
      frame 7 {
        w250 = 1.0
        w242 = "my_blackboard" ("Blackboard name")
        # "Read after Shutdown"
        n106 = call "Initialize.vi"("error in (no error)"=w259, "Node name"="my_node") -> ("error out"=w260:errorcluster)  [unwired: 9 in]
        n107 = call "Create Blackboard.vi"("error in (no error)"=w260, "Blackboard name"=w242) -> ("error out"=w257:errorcluster, "Blackboard Reference"=w254:T3)  [unwired: 8 in]
        n108 = Bundle By Name(cluster=T1 {"BlackBoard"="", "Topic"="my_data", "Type Override"=""} ("Topic Full Names"), "BlackBoard"=w242) -> (w241:T1)
        n109 = call "Create Writer.vim"("error in (no error)"=w257, "Data"=w250, "Topic Name"=w241, "BlackBoard Reference"=w254) -> ("error out"=w258:errorcluster)  [unwired: 5 in, 2 out]
        n110 = call "Start Blackboard.vi"("error in (no error)"=w258, "Blackboard Reference"=w254) -> ("error out"=w256:errorcluster)  [unwired: 9 in]
        n111 = call "Create Reader.vim"("error in (no error)"=w256, "Data Type"=w250, "Topic Name"=w241) -> ("error out"=w251:errorcluster, "Reader Reference"=w253:T5)  [unwired: 6 in, 1 out]
        n112 = call "Destroy Blackboard.vi"("error in (no error)"=w251, "Blackboard Reference"=w254) -> ("error out"=w249:errorcluster)  [unwired: 8 in, 1 out]
        n113 = call "Shutdown Iceoryx.vi"("error in (no error)"=w249) -> ("error out"=w248:errorcluster)  [unwired: 10 in]
        n114 = call "Read.vim"("error in (no error)"=w248, "Data In"=w250, "Reader Reference"=w253) -> ("error out"=w252:errorcluster)  [unwired: 6 in, 2 out]
        n115 = call "Destroy Reader.vim"("error in (no error)"=w252, "Reader Reference"=w253) -> ("error out"=w247:errorcluster)  [unwired: 9 in]
        n116 = call <vilib>:"Clear Errors.vi"("error in (no error)"=w247, "specific error code to clear (0: all)"=8101) -> ("error out"=w246:errorcluster, "specific error cleared?"=w244:bool)  [unwired: 4 in]
        n117 = Compound Arithmetic op=AND(invert w246, w244) -> (w261:bool)
        n118 = case shown="False" w261 {
          tunnel: w265 -> [w269 w270]
          tunnel: [w266 w270] -> w264
          tunnel: "Failed read after Shutdown" -> [w268 _]
          tunnel: "\r" -> [w267 _]
          frame False {
            n119 = Concatenate Strings(w269, w268, w267) -> (w266:string)
          }
          frame True {
          }
        }
      }
      frame 8 {
        w282 = 1.0
        w273 = "my_blackboard" ("Blackboard name")
        # "Write after Shutdown"
        n120 = call "Initialize.vi"("error in (no error)"=w291, "Node name"="my_node") -> ("error out"=w292:errorcluster)  [unwired: 9 in]
        n121 = call "Create Blackboard.vi"("error in (no error)"=w292, "Blackboard name"=w273) -> ("error out"=w289:errorcluster, "Blackboard Reference"=w286:T3)  [unwired: 8 in]
        n122 = Bundle By Name(cluster=T1 {"BlackBoard"="", "Topic"="my_data", "Type Override"=""} ("Topic Full Names"), "BlackBoard"=w273) -> (w272:T1)
        n123 = call "Create Writer.vim"("error in (no error)"=w289, "Data"=w282, "Topic Name"=w272, "BlackBoard Reference"=w286) -> ("error out"=w290:errorcluster, "Writer Reference"=w275:T4)  [unwired: 5 in, 1 out]
        n124 = call "Start Blackboard.vi"("error in (no error)"=w290, "Blackboard Reference"=w286) -> ("error out"=w288:errorcluster)  [unwired: 9 in]
        n125 = call "Create Reader.vim"("error in (no error)"=w288, "Data Type"=w282, "Topic Name"=w272) -> ("error out"=w283:errorcluster, "Reader Reference"=w285:T5)  [unwired: 6 in, 1 out]
        n126 = call "Destroy Blackboard.vi"("error in (no error)"=w283, "Blackboard Reference"=w286) -> ("error out"=w281:errorcluster)  [unwired: 8 in, 1 out]
        n127 = call "Shutdown Iceoryx.vi"("error in (no error)"=w281) -> ("error out"=w280:errorcluster)  [unwired: 10 in]
        n128 = call "Write.vim"("error in (no error)"=w280, "Data In"=1.0, "Writer Reference"=w275) -> ("error out"=w284:errorcluster)  [unwired: 7 in, 1 out]
        n129 = call "Destroy Reader.vim"("error in (no error)"=w284, "Reader Reference"=w285) -> ("error out"=w279:errorcluster)  [unwired: 9 in]
        n130 = call <vilib>:"Clear Errors.vi"("error in (no error)"=w279, "specific error code to clear (0: all)"=8101) -> ("error out"=w278:errorcluster, "specific error cleared?"=w276:bool)  [unwired: 4 in]
        n131 = Compound Arithmetic op=AND(invert w278, w276) -> (w293:bool)
        n132 = case shown="False" w293 {
          tunnel: w297 -> [w301 w302]
          tunnel: [w298 w302] -> w296
          tunnel: "Failed write after Shutdown" -> [w300 _]
          tunnel: "\r" -> [w299 _]
          frame False {
            n133 = Concatenate Strings(w301, w300, w299) -> (w298:string)
          }
          frame True {
          }
        }
      }
      frame 9 {
        w314 = dbl[] [1.0, 6.28, 0.0, 0.0, 0.0, 0.0, 7.0, 3.14]
        w304 = "my_blackboard" ("Blackboard name")
        # "Read partial"
        n134 = call "Initialize.vi"("error in (no error)"=w320, "Node name"="my_node") -> ("error out"=w332:errorcluster)  [unwired: 9 in]
        n135 = call "Create Blackboard.vi"("error in (no error)"=w332, "Blackboard name"=w304) -> ("error out"=w330:errorcluster, "Blackboard Reference"=w321:T3)  [unwired: 8 in]
        n136 = Bundle By Name(cluster=T1 {"BlackBoard"="", "Topic"="my_data", "Type Override"="Array1"} ("Topic Full Names"), "BlackBoard"=w304) -> (w303:T1)
        n137 = call "Create Writer.vim"("error in (no error)"=w330, "Data"=dbl[] [0.0, 0.0, 0.0, 0.0, 0.0, 0.0, 7.0, 8.0], "Topic Name"=w303, "BlackBoard Reference"=w321) -> ("error out"=w331:errorcluster, "Writer Reference"=w323:T4)  [unwired: 5 in, 1 out]
        n138 = call "Start Blackboard.vi"("error in (no error)"=w331, "Blackboard Reference"=w321) -> ("error out"=w329:errorcluster)  [unwired: 9 in]
        n139 = call "Create Raw Reader.vi"("error in (no error)"=w329, "Topic Full Names"=w303) -> ("error out"=w328:errorcluster, "Raw Reader Reference"=w322:T7)  [unwired: 8 in]
        n140 = Index Array(array=w314, index=1) -> (element=w312:dbl)
        n141 = call "Write.vim"("error in (no error)"=w328, "Data In"=w314, "Writer Reference"=w323) -> ("error out"=w327:errorcluster)  [unwired: 7 in, 1 out]
        n142 = call "Read Partial Raw.vi"("error in (no error)"=w327, "Read Offset (bytes)"=u32 16, "Data In"=u8[] [0, 0, 0, 0, 0, 0, 0, 0], "Raw Reader Reference"=w322) -> ("error out"=w326:errorcluster, "Data Length"=w310:u32, "Data Out"=w316:u8[])  [unwired: 5 in]
        n143 = call "Unflatten Structure from U8.vim"("Type"=w312, "Flattend Data in"=w316) -> ("Unflattend Data"=w311:dbl)  [unwired: 7 in, 2 out]
        n144 = call "Destroy Reader.vim"("error in (no error)"=w326, "Reader Reference"=w322) -> ("error out"=w325:errorcluster)  [unwired: 9 in]
        n145 = Equal?(x=w310, y=u32 8) -> (x = y?=w308:bool)
        n146 = Equal?(x=w311, y=w312) -> (x = y?=w307:bool)
        n147 = call "Destroy Blackboard.vi"("error in (no error)"=w325, "Blackboard Reference"=w321) -> ("error out"=w319:errorcluster)  [unwired: 8 in, 1 out]
        n148 = Compound Arithmetic op=AND(invert w319, w308, w307) -> (w318:bool)
        n149 = case shown="True" w318 {
          tunnel: w336 -> [w340 w341]
          tunnel: [w337 w341] -> w335
          tunnel: "Failed partial read" -> [w339 _]
          tunnel: "\r" -> [w338 _]
          frame False {
            n150 = Concatenate Strings(w340, w339, w338) -> (w337:string)
          }
          frame True {
          }
        }
      }
      frame 10 {
        w347 = 314
        w343 = "my_blackboard" ("Blackboard name")
        # "Automatic conversion"
        n151 = call "Initialize.vi"("error in (no error)"=w363, "Node name"="my_node") -> ("error out"=w364:errorcluster)  [unwired: 9 in]
        n152 = call "Create Blackboard.vi"("error in (no error)"=w364, "Blackboard name"=w343) -> ("error out"=w361:errorcluster, "Blackboard Reference"=w353:T3)  [unwired: 8 in]
        n153 = Bundle By Name(cluster=T1 {"BlackBoard"="", "Topic"="my_data", "Type Override"=""} ("Topic Full Names"), "BlackBoard"=w343) -> (w342:T1)
        n154 = call "Create Writer.vim"("error in (no error)"=w361, "Data"=0, "Topic Name"=w342, "BlackBoard Reference"=w353) -> ("error out"=w362:errorcluster, "Writer Reference"=w355:T4)  [unwired: 5 in, 1 out]
        n155 = call "Start Blackboard.vi"("error in (no error)"=w362, "Blackboard Reference"=w353) -> ("error out"=w360:errorcluster)  [unwired: 9 in]
        n156 = call "Create Reader.vim"("error in (no error)"=w360, "Data Type"=0.0, "Topic Name"=w342) -> ("error out"=w359:errorcluster, "Reader Reference"=w354:T5)  [unwired: 6 in, 1 out]
        n157 = call "Write.vim"("error in (no error)"=w359, "Data In"=w347, "Writer Reference"=w355) -> ("error out"=w358:errorcluster)  [unwired: 7 in, 1 out]
        n158 = To Double Precision Float(number=w347) -> (double precision float=w346:dbl)
        n159 = call "Read.vim"("error in (no error)"=w358, "Data In"=0.0, "Reader Reference"=w354) -> ("error out"=w349:errorcluster, "Data Out"=w351:dbl)  [unwired: 6 in, 1 out]
        n160 = Equal?(x=w351, y=w346) -> (x = y?=w365:bool)
        n161 = call "Destroy Reader.vim"("error in (no error)"=w349, "Reader Reference"=w354) -> ("error out"=w357:errorcluster)  [unwired: 9 in]
        n162 = call "Destroy Blackboard.vi"("error in (no error)"=w357, "Blackboard Reference"=w353) -> ("error out"=w350:errorcluster)  [unwired: 8 in, 1 out]
        n163 = Compound Arithmetic op=AND(invert w350, w365) -> (w366:bool)
        n164 = case shown="True" w366 {
          tunnel: w370 -> [w374 w375]
          tunnel: [w371 w375] -> w369
          tunnel: "Failed data conversion" -> [w373 _]
          tunnel: "\r" -> [w372 _]
          frame False {
            n165 = Concatenate Strings(w374, w373, w372) -> (w371:string)
          }
          frame True {
          }
        }
      }
      frame 11 {
        w383 = T2 {"U16"=0, "test_I32"=314, TRUE, "embedded"={0.0, "bool"=FALSE}}
        w376 = "my_blackboard" ("Blackboard name")
        # "Cluster Element Read"
        n166 = call "Initialize.vi"("error in (no error)"=w400, "Node name"="my_node") -> ("error out"=w401:errorcluster)  [unwired: 9 in]
        n167 = call "Create Blackboard.vi"("error in (no error)"=w401, "Blackboard name"=w376) -> ("error out"=w398:errorcluster, "Blackboard Reference"=w391:T3)  [unwired: 8 in]
        n168 = Bundle By Name(cluster=T1 {"BlackBoard"="", "Topic"="my_data", "Type Override"="My_Cluster"} ("Topic Full Names"), "BlackBoard"=w376) -> (w379:T1)
        n169 = call "Create Writer.vim"("error in (no error)"=w398, "Data"=T2 {"U16"=0, "test_I32"=0, TRUE, "embedded"={0.0, "bool"=FALSE}}, "Topic Name"=w379, "BlackBoard Reference"=w391) -> ("error out"=w399:errorcluster, "Writer Reference"=w393:T4)  [unwired: 5 in, 1 out]
        n170 = Bundle By Name(cluster=T1 {"BlackBoard"="", "Topic"="my_data.test_I32", "Type Override"=""} ("Topic Full Names"), "BlackBoard"=w376) -> (w378:T1)
        n171 = call "Start Blackboard.vi"("error in (no error)"=w399, "Blackboard Reference"=w391) -> ("error out"=w381:errorcluster)  [unwired: 9 in]
        n172 = call "Create Reader.vim"("error in (no error)"=w381, "Data Type"=0.0, "Topic Name"=w378) -> ("error out"=w397:errorcluster, "Reader Reference"=w392:T5)  [unwired: 6 in, 1 out]
        n173 = call "Write.vim"("error in (no error)"=w397, "Data In"=w383, "Writer Reference"=w393) -> ("error out"=w396:errorcluster)  [unwired: 7 in, 1 out]
        n174 = Unbundle By Name(w383) -> ("test_I32"=w382:i32)
        n175 = To Double Precision Float(number=w382) -> (double precision float=w386:dbl)
        n176 = call "Read.vim"("error in (no error)"=w396, "Data In"=0.0, "Reader Reference"=w392) -> ("error out"=w388:errorcluster, "Data Out"=w390:dbl)  [unwired: 6 in, 1 out]
        n177 = Equal?(x=w390, y=w386) -> (x = y?=w402:bool)
        n178 = call "Destroy Reader.vim"("error in (no error)"=w388, "Reader Reference"=w392) -> ("error out"=w395:errorcluster)  [unwired: 9 in]
        n179 = call "Destroy Blackboard.vi"("error in (no error)"=w395, "Blackboard Reference"=w391) -> ("error out"=w389:errorcluster)  [unwired: 8 in, 1 out]
        n180 = Compound Arithmetic op=AND(invert w389, w402) -> (w403:bool)
        n181 = case shown="True" w403 {
          tunnel: w407 -> [w411 w412]
          tunnel: [w408 w412] -> w406
          tunnel: "Failed data conversion" -> [w410 _]
          tunnel: "\r" -> [w409 _]
          frame False {
            n182 = Concatenate Strings(w411, w410, w409) -> (w408:string)
          }
          frame True {
          }
        }
      }
      frame 12 {
        w423 = "my_blackboard" ("Blackboard name")
        # "Read Descriptor"
        n183 = call "Initialize.vi"("error in (no error)"=w430, "Node name"="my_node") -> ("error out"=w431:errorcluster)  [unwired: 9 in]
        n184 = call "Create Blackboard.vi"("error in (no error)"=w431, "Blackboard name"=w423) -> ("error out"=w428:errorcluster, "Blackboard Reference"=w426:T3)  [unwired: 8 in]
        n185 = Bundle By Name(cluster=T1 {"BlackBoard"="", "Topic"="my_data", "Type Override"="My_Cluster"} ("Topic Full Names"), "BlackBoard"=w423) -> (w419:T1)
        n186 = call "Create Writer.vim"("error in (no error)"=w428, "Data"=T2 {"U16"=0, "test_I32"=0, TRUE, "embedded"={0.0, "bool"=FALSE}}, "Topic Name"=w419, "BlackBoard Reference"=w426) -> ("error out"=w429:errorcluster)  [unwired: 5 in, 2 out]
        n187 = call "Start Blackboard.vi"("error in (no error)"=w429, "Blackboard Reference"=w426) -> ("error out"=w421:errorcluster)  [unwired: 9 in]
        n188 = call "Read Topic Descriptor.vi"("error in (no error)"=w421, "Topic Full Names"=w419) -> ("error out"=w420:errorcluster, "type_name"=w417:string, "descriptor"=w415:string)  [unwired: 7 in]
        n189 = Equal?(x=w417, y="My_Cluster" ("type_name")) -> (x = y?=w414:bool)
        n190 = Equal?(x=w415, y="{ \"endianness\": \"little\", \"array\": false, \"arraysize\": 1, \"elemsize\" : 32, \"struct_elems\" : [{ \"name\": \"U16\", \"type\": \"u16\", \"size\": 2, \"offset\": 0},{ \"name\": \"test_I32\", \"type\": \"i32\", \"size\": 4, \"offset\": 4},{ \"name\": \"Boolean\", \"type\": \"bool\", \"size\": 1, \"offset\": 8},{ \"name\": \"embedded.DoubleFloat\", \"type\": \"f64\", \"size\": 8, \"offset\": 16},{ \"name\": \"embedded.bool\", \"type\": \"bool\", \"size\": 1, \"offset\": 24}] }" ("descriptor 2")) -> (x = y?=w413:bool)
        n191 = call "Destroy Blackboard.vi"("error in (no error)"=w420, "Blackboard Reference"=w426) -> ("error out"=w425:errorcluster)  [unwired: 8 in, 1 out]
        n192 = Compound Arithmetic op=AND(invert w425, w414, w413) -> (w432:bool)
        n193 = case shown="True" w432 {
          tunnel: w436 -> [w440 w441]
          tunnel: [w437 w441] -> w435
          tunnel: "Failed read descriptor" -> [w439 _]
          tunnel: "\r" -> [w438 _]
          frame False {
            n194 = Concatenate Strings(w440, w439, w438) -> (w437:string)
          }
          frame True {
          }
        }
      }
      frame 13 {
        w445 = dbl[] [0.0, 0.0, 0.0, 0.0, 0.0, 0.0, 7.0, 8.0]
        w456 = "my_blackboard" ("Blackboard name")
        # "8 elements plus the 8 byte size header"
        # "Read Size"
        n195 = call "Initialize.vi"("error in (no error)"=w460, "Node name"="my_node") -> ("error out"=w467:errorcluster)  [unwired: 9 in]
        n196 = call "Create Blackboard.vi"("error in (no error)"=w467, "Blackboard name"=w456) -> ("error out"=w465:errorcluster, "Blackboard Reference"=w461:T3)  [unwired: 8 in]
        n197 = Bundle By Name(cluster=T1 {"BlackBoard"="", "Topic"="my_data", "Type Override"="Array1"} ("Topic Full Names"), "BlackBoard"=w456) -> (w454:T1)
        n198 = call "Create Writer.vim"("error in (no error)"=w465, "Data"=w445, "Topic Name"=w454, "BlackBoard Reference"=w461) -> ("error out"=w466:errorcluster)  [unwired: 5 in, 2 out]
        n199 = call "Start Blackboard.vi"("error in (no error)"=w466, "Blackboard Reference"=w461) -> ("error out"=w464:errorcluster)  [unwired: 9 in]
        n200 = call "Create Raw Reader.vi"("error in (no error)"=w464, "Topic Full Names"=w454) -> ("error out"=w455:errorcluster, "Raw Reader Reference"=w453:T7)  [unwired: 8 in]
        n201 = call "Create Reader.vim"("error in (no error)"=w455, "Data Type"=w445, "Topic Name"=w454) -> ("error out"=w452:errorcluster, "Reader Reference"=w450:T5)  [unwired: 6 in, 1 out]
        n202 = call "Read Raw Size.vim"("error in (no error)"=w452, "Raw Reader Reference"=w453) -> ("error out"=w451:errorcluster, "Max Bytes"=w444:u32)  [unwired: 8 in]
        n203 = call "Read Raw Size.vim"("error in (no error)"=w451, "Raw Reader Reference"=w450) -> ("error out"=w449:errorcluster, "Max Bytes"=w447:u32)  [unwired: 8 in]
        n204 = Equal?(x=w447, y=w444) -> (x = y?=w446:bool)
        n205 = Equal?(x=w444, y=u32 72) -> (x = y?=w442:bool)
        n206 = call "Destroy Reader.vim"("error in (no error)"=w449, "Reader Reference"=w450) -> ("error out"=w448:errorcluster)  [unwired: 9 in]
        n207 = call "Destroy Reader.vim"("error in (no error)"=w448, "Reader Reference"=w453) -> ("error out"=w463:errorcluster)  [unwired: 9 in]
        n208 = call "Destroy Blackboard.vi"("error in (no error)"=w463, "Blackboard Reference"=w461) -> ("error out"=w459:errorcluster)  [unwired: 8 in, 1 out]
        n209 = Compound Arithmetic op=AND(invert w459, w446, w442) -> (w458:bool)
        n210 = case shown="True" w458 {
          tunnel: w471 -> [w475 w476]
          tunnel: [w472 w476] -> w470
          tunnel: "Failed Read Size" -> [w474 _]
          tunnel: "\r" -> [w473 _]
          frame False {
            n211 = Concatenate Strings(w475, w474, w473) -> (w472:string)
          }
          frame True {
          }
        }
      }
      frame 14 {
        w483 = u8[] [1, 0, 0, 0, 0, 0, 7, 3]
        w479 = "my_blackboard" ("Blackboard name")
        # "Write and Read Raw"
        n212 = call "Initialize.vi"("error in (no error)"=w487, "Node name"="my_node") -> ("error out"=w498:errorcluster)  [unwired: 9 in]
        n213 = call "Create Blackboard.vi"("error in (no error)"=w498, "Blackboard name"=w479) -> ("error out"=w478:errorcluster, "Blackboard Reference"=w488:T3)  [unwired: 8 in]
        n214 = Bundle By Name(cluster=T1 {"BlackBoard"="", "Topic"="my_data", "Type Override"="Array1"} ("Topic Full Names"), "BlackBoard"=w479) -> (w477:T1)
        n215 = call "Create Raw Writer.vi"("error in (no error)"=w478, "Data"=u8[] [0, 0, 0, 0, 0, 0, 7, 8], "Topic Name"=w477, "BlackBoard Reference"=w488) -> ("error out"=w497:errorcluster, "Raw Writer Reference"=w490:T8)  [unwired: 5 in, 1 out]
        n216 = call "Start Blackboard.vi"("error in (no error)"=w497, "Blackboard Reference"=w488) -> ("error out"=w496:errorcluster)  [unwired: 9 in]
        n217 = call "Create Raw Reader.vi"("error in (no error)"=w496, "Topic Full Names"=w477) -> ("error out"=w495:errorcluster, "Raw Reader Reference"=w489:T7)  [unwired: 8 in]
        n218 = call "Write Raw.vi"("error in (no error)"=w495, "Data In"=w483, "Writer Reference"=w490) -> ("error out"=w494:errorcluster)  [unwired: 7 in, 1 out]
        n219 = call "Read Raw.vi"("error in (no error)"=w494, "Data In"=u8[] [0, 0, 0, 0, 0, 0, 7, 8], "Raw Reader Reference"=w489) -> ("error out"=w493:errorcluster, "Data Out"=w482:u8[])  [unwired: 5 in, 2 out]
        n220 = Equal?(x=w482, y=w483) -> (x = y?=w499:bool)
        n221 = call "Destroy Reader.vim"("error in (no error)"=w493, "Reader Reference"=w489) -> ("error out"=w492:errorcluster)  [unwired: 9 in]
        n222 = call "Destroy Blackboard.vi"("error in (no error)"=w492, "Blackboard Reference"=w488) -> ("error out"=w486:errorcluster)  [unwired: 8 in, 1 out]
        n223 = Compound Arithmetic op=AND(invert w486, w499) -> (w485:bool)
        n224 = case shown="True" w485 {
          tunnel: w503 -> [w507 w508]
          tunnel: [w504 w508] -> w502
          tunnel: "Failed Write and Read Raw" -> [w506 _]
          tunnel: "\r" -> [w505 _]
          frame False {
            n225 = Concatenate Strings(w507, w506, w505) -> (w504:string)
          }
          frame True {
          }
        }
      }
    }
  }
  "error out" <- w1
  "status" <- w3
  n226 = And Array Elements(Boolean array=w7) -> (logical AND=→"pass":bool)
